vi "PageExplorer_Global_Init.vi"(11 "Object":T1) -> ()   [LabVIEW 2020]
uses:
  <resource>/Framework/Providers/API/ItemRef.ctl
  <resource>/dialog/lvconfig.llb/LV Config Read Boolean.vi
panel:
  out "error out":errorcluster
  in  "error in":errorcluster
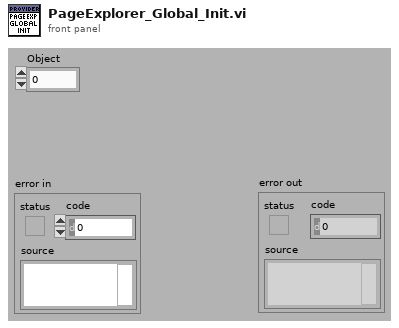
[diagram p1: front panel]
types:
  T1 = typedef "ItemRef.ctl" = u64
  T2 = enum32{"Invalid", "Standard", "Closed", "Hidden", "Minimized", "Maximized"}
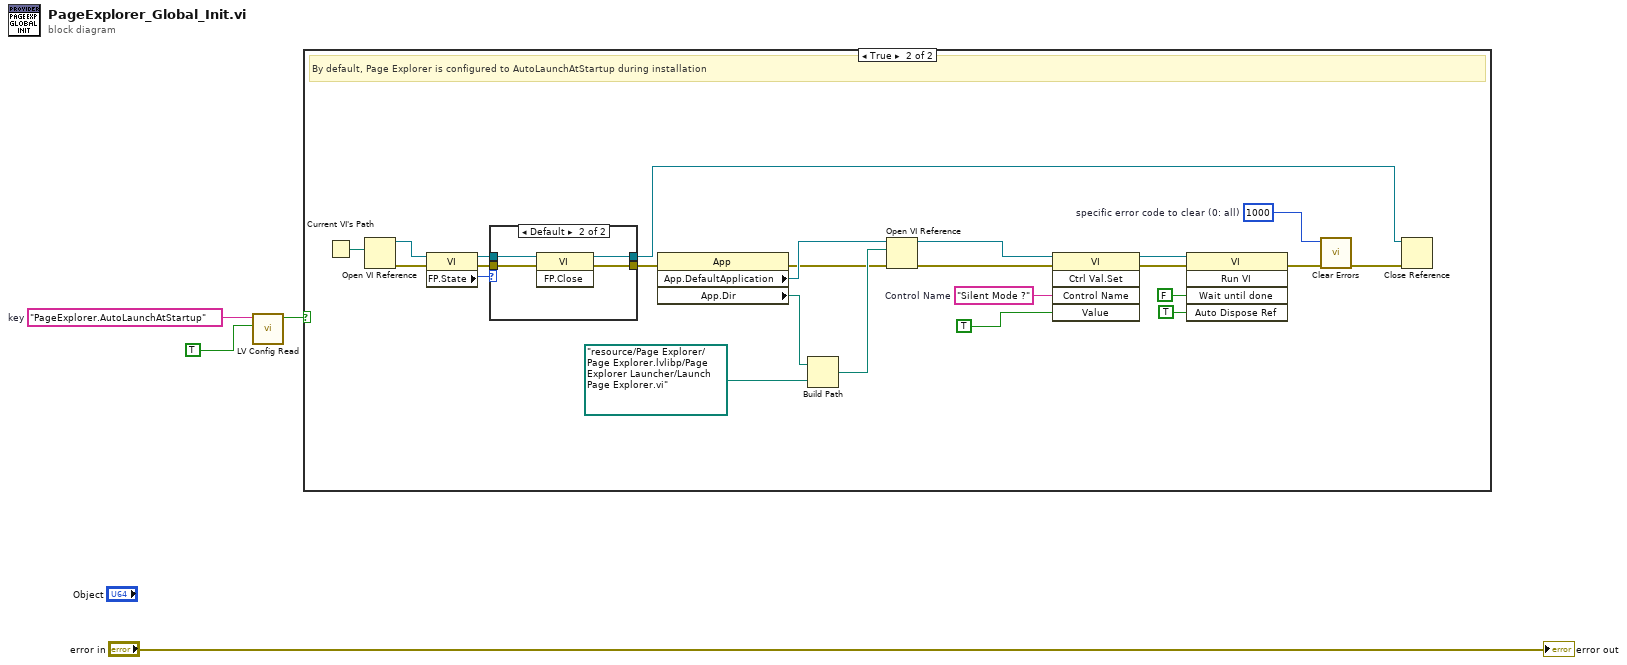
[diagram p0: block diagram]
diagram:
  w2 = "PageExplorer.AutoLaunchAtStartup"  # key
  n1 = call-poly <resource>:"LV Config Read.vi"("default value"=TRUE, "key"=w2) -> ("value"=w3:bool)  [unwired: 3 in, 2 out]
  n2 = case shown="True" w3 {
    frame False {
    }
    frame True {
      w10 = "Silent Mode ?"  # Control Name
      w11 = 1000  # specific error code to clear (0: all)
      # "By default, Page Explorer is configured to AutoLaunchAtStartup during installation"
      n3 = Current VI's Path() -> (path=w22:path)
      n4 = Open VI Reference(vi path=w22) -> (vi reference=w19:refnum<vi>, error out=w18:errorcluster)  [unwired: 5 in]
      n5 = property class="VI"(reference=w19, error in=w18) -> (reference out=w20:refnum<vi>, error out=w21:errorcluster, "FP.State"=w17:T2)
      n6 = case shown="Default" w17 {
        tunnel: [w30 w34] -> w16
        tunnel: w21 -> [w30 w33]
        tunnel: w20 -> [w29 w32]
        tunnel: [w29 w31] -> w15
        frame "Invalid", "Closed" {
        }
        frame Default {
          n7 = invoke class="VI" method="FP.Close"(reference=w32, error in=w33) -> (reference out=w31:refnum<vi>, error out=w34:errorcluster)  [unwired: 1 in, 1 out]
        }
      }
      n8 = property class="App"(error in=w16) -> (error out=w24:errorcluster, "App.DefaultApplication"=w25:refnum<vi>, "App.Dir"=w28:path)  [unwired: 1 in, 1 out]
      n9 = Build Path(base path=w28, name or relative path=path "resource/Page Explorer/Page Explorer.lvlibp/Page Explorer Launcher/Launch Page Explorer.vi" ("vi path")) -> (appended path=w26:path)
      n10 = Open VI Reference(application reference (local)=w25, vi path=w26, error in (no error)=w24) -> (vi reference=w6:refnum<vi>, error out=w5:errorcluster)  [unwired: 3 in]
      n11 = invoke class="VI" method="Ctrl Val.Set"(reference=w6, error in=w5, "Control Name"=w10, "Value"=TRUE ("Auto Dispose Reference")) -> (reference out=w7:refnum<vi>, error out=w8:errorcluster)  [unwired: 1 in, 3 out]
      n12 = invoke class="VI" method="Run VI"(reference=w7, error in=w8, "Wait until done"=FALSE ("Wait Until Done"), "Auto Dispose Ref"=TRUE ("Auto Dispose Reference")) -> (error out=w12:errorcluster)  [unwired: 1 in, 4 out]
      n13 = call <vilib>:"Clear Errors.vi"("error in (no error)"=w12, "specific error code to clear (0: all)"=w11) -> ("error out"=w23:errorcluster)  [unwired: 4 in, 1 out]
      n14 = Close Reference(reference=w15, error in (no error)=w23) -> ()  [unwired: 1 out]
    }
  }
  "error out" <- "error in"
